vi "Userstep_allstepspath.vi"() -> (3 "Array":path[](array[path]))   [LabVIEW 2017, in "NLTest.lvclass"]
uses:
  NLTest.lvclass
panel:
  in  "Listbox":i32(listbox)
  # "有新的子项，重命名，\n记得运行并保存这个VI！\n此输出userstep"
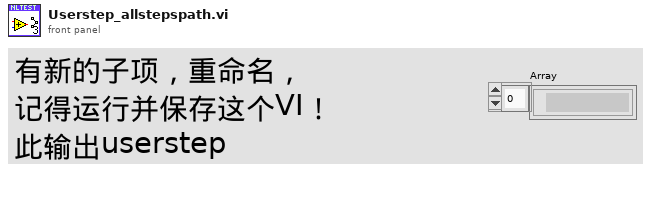
[diagram p1: front panel]
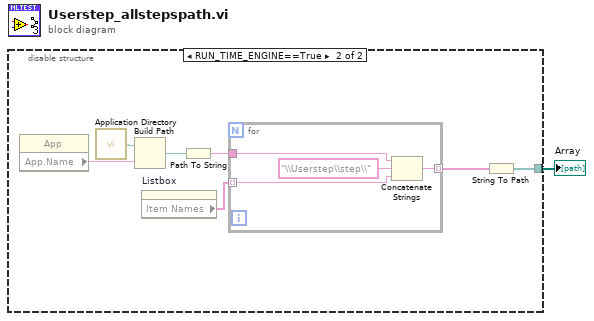
[diagram p0: block diagram]
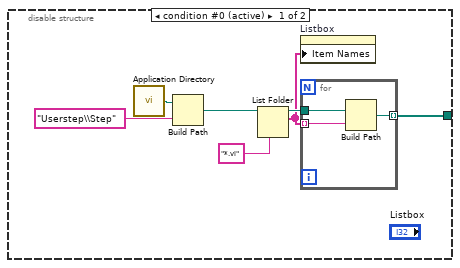
[diagram p2: hidden frame]
diagram:
  n1 = disable-structure shown="RUN_TIME_ENGINE==True" {
    disable-tunnel: [w2 w12] -> w1
    frame condition #0 (active) {
      n2 = call <vilib>:"Application Directory.vi"() -> ("Application Directory"=w8:path)
      n3 = Build Path(base path=w8, name or relative path="Userstep\\Step") -> (appended path=w6:path)
      n4 = List Folder(path=w6, pattern="*.vi") -> (path out=w4:path, filenames=w3:string[])  [unwired: 2 in, 2 out]
      n5 = property on="Listbox" class="LstBox (strict)"("Item Names"=w3) -> ()  [unwired: 2 in, 2 out]
      n6 = for {
        tunnel: w4 -> [w11]
        tunnel: w3 -> [w10] mode=indexing
        tunnel: [w9] -> w2 mode=indexing
        n7 = Build Path(base path=w11, name or relative path=w10) -> (appended path=w9:path)
      }
    }
    frame condition #1 {
      n8 = property class="App"() -> ("App.Name"=w17:string)  [unwired: 2 in, 2 out]
      n9 = call <vilib>:"Application Directory.vi"() -> ("Application Directory"=w18:path)
      n10 = Build Path(base path=w18, name or relative path=w17) -> (appended path=w16:path)
      n11 = property on="Listbox" class="LstBox (strict)"() -> ("Item Names"=w14:string[])  [unwired: 2 in, 2 out]
      n12 = Path To String(path=w16) -> (string=w15:string)
      n13 = for {
        tunnel: w15 -> [w22]
        tunnel: w14 -> [w20] mode=indexing
        tunnel: [w19] -> w13 mode=indexing
        n14 = Concatenate Strings(w22, "\\Userstep\\step\\", w20) -> (w19:string)
      }
      n15 = String To Path(string=w13) -> (path=w12:path[])
    }
  }
  "Array" <- w1
